vi "Read.vi"(0 "UCI_DllPath":path, 1 "Command":string="mea:all?;", 2 "Session_id":u32, 3 "Length":u32=400, 4 "Timeout":u32=2000, 5 "InputData":u8[](array[numeric])) -> (6 "OutputData":u8[](array[numeric]), 7 "Result":i32, 8 "ResultDescription":string)   [LabVIEW 2015]
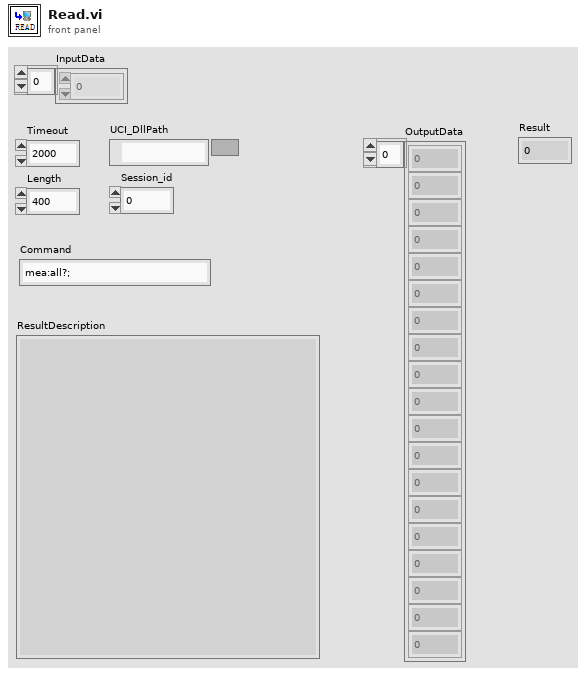
[diagram p1: front panel]
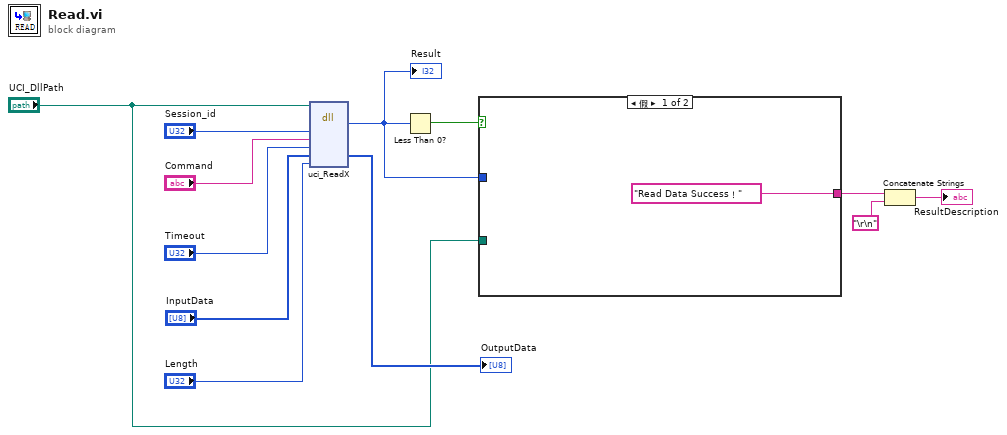
[diagram p0: block diagram]
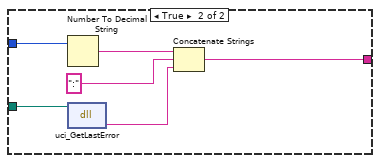
[diagram p2: hidden frame]
diagram:
  n1 = dll-call lib="E:/JL-Project/LabView-Project/ASCII/uci.dll" fn="uci_ReadX"(path in="UCI_DllPath", "session"="Session_id", "msg"="Command", "timeout"="Timeout", "data"="InputData", "len"="Length") -> ("返回类型"=w9:i32, "data"=→"OutputData":u8[])  [unwired: 6 in, 2 out]
  "Result" <- w9
  n2 = Less Than 0?(x=w9) -> (x < 0?=w10:bool)
  n3 = case shown="假" w10 {
    tunnel: w9 -> [_ w16]
    tunnel: "UCI_DllPath" -> [_ w15]
    tunnel: ["Read Data Success！" w14] -> w2
    frame False {
    }
    frame True {
      n4 = Number To Decimal String(number=w16) -> (decimal integer string=w17:string)  [unwired: 1 in]
      n5 = dll-call lib="E:/JL-Project/LabView-Project/ASCII/uci.dll" fn="uci_GetLastError"(path in=w15) -> ("返回类型"=w19:string)  [unwired: 2 in, 2 out]
      n6 = Concatenate Strings(w17, ":" ("字符串"), w19) -> (w14:string)
    }
  }
  n7 = Concatenate Strings(w2, "\r\n") -> (→"ResultDescription":string)
